vi "Own20261012_PublicAddRootDecoration_v2.vi"() -> ()   [LabVIEW 2024]
panel:
  out "error out":errorcluster caption="错误输出"
  out "object_id":u32
  in  "object_id type":u32
  in  "y":i16=100
  in  "x":i16=100
  in  "style":u32
  in  "target_path":path
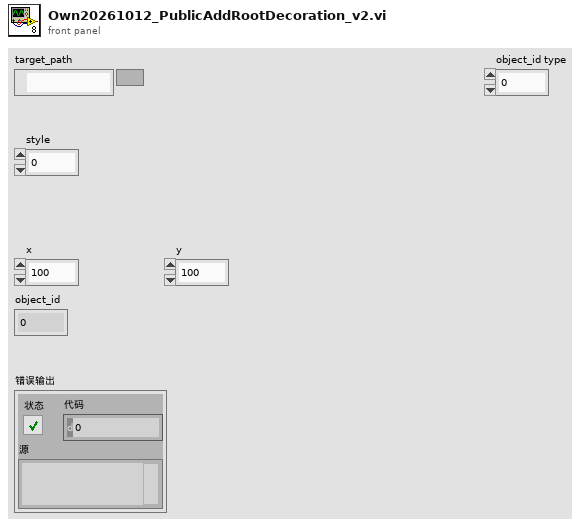
[diagram p1: front panel]
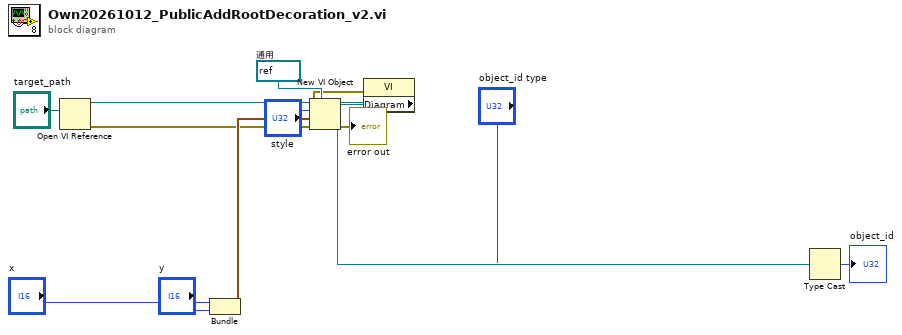
[diagram p0: block diagram]
diagram:
  w13 = refnum<vi> refnum  # 通用
  n1 = Open VI Reference ("打开VI引用")(vi path="target_path") -> (vi reference=w4:refnum<vi>, error out=w3:errorcluster)  [unwired: 5 in]
  n2 = Bundle ("捆绑")("x"="x", "y"="y") -> (w9:cluster{"x":i16, "y":i16})  [unwired: 1 in]
  n3 = property class="VI"(reference=w4, error in=w3) -> (error out=w1:errorcluster, "Diagram"=w2:refnum<vi>)  [unwired: 1 out]
  n4 = New VI Object ("新建VI对象")(vi object class=w13, owner refnum=w2, style="style", position/next to=w9, 8:w1) -> (object refnum=w8:refnum<vi>, 0:→"error out":errorcluster)  [unwired: 3 in]
  n5 = Type Cast ("强制类型转换")(type="object_id type", x=w8) -> (*(type *) &x=→"object_id":u32)
